vi "ingest.video-with_manifest_timestamp.vi"(6 "Properties and Labels":T1, 7 "Timestamp S3 Path":string, 8 "error in":errorcluster, 9 "Title and Description":cluster{"Title":string, "Description":string}, 10 "S3 Path":string, 11 "Nominal Client in":refnum<class "Nominal Client.lvclass">) -> (0 "error out":errorcluster, 1 "Response":T2, 2 "Video RID":string, 3 "Nominal Client out":refnum<class "Nominal Client.lvclass">, 4 "Response":string)   [LabVIEW 2020, in "Nominal Client.lvclass"]
doc: "Ingests video data from a S3 Nominal upload bucket."
uses:
  Nominal Client.lvclass
  4b965f09-dc68-4d5e-a5c1-32d476accfd4.vi
  1697451f-e5b3-4789-844d-430f2d519a58.vi
  bab285cf-d058-4520-b957-25c58aac0c58.vi
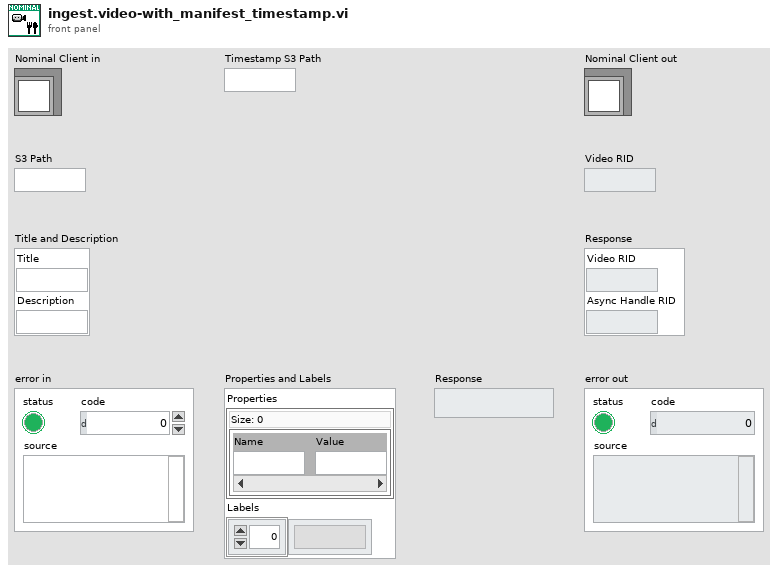
[diagram p1: front panel]
types:
  T1 = cluster{"Properties":map{string, string}, "Labels":string[]}
  T2 = cluster{"Video RID":string, "Async Handle RID":string}
  T3 = cluster{"type":string, "s3":cluster{"path":string}}[]
  T4 = cluster{"type":string, "s3":cluster{"path":string}}
  T5 = cluster{"type":string, "timestampManifests":cluster{"sources":cluster{"type":string, "s3":cluster{"path":string}}[]}}
  T6 = cluster{"videoRid":string, "asyncHandle":cluster{"rid":string}}
  T7 = cluster{"sources":cluster{"type":string, "s3":cluster{"path":string}}[], "properties":string, "labels":string[], "timestamps":cluster{"type":string, "timestampManifests":cluster{"sources":cluster{"type":string, "s3":cluster{"path":string}}[]}}, "title":string, "description":string}
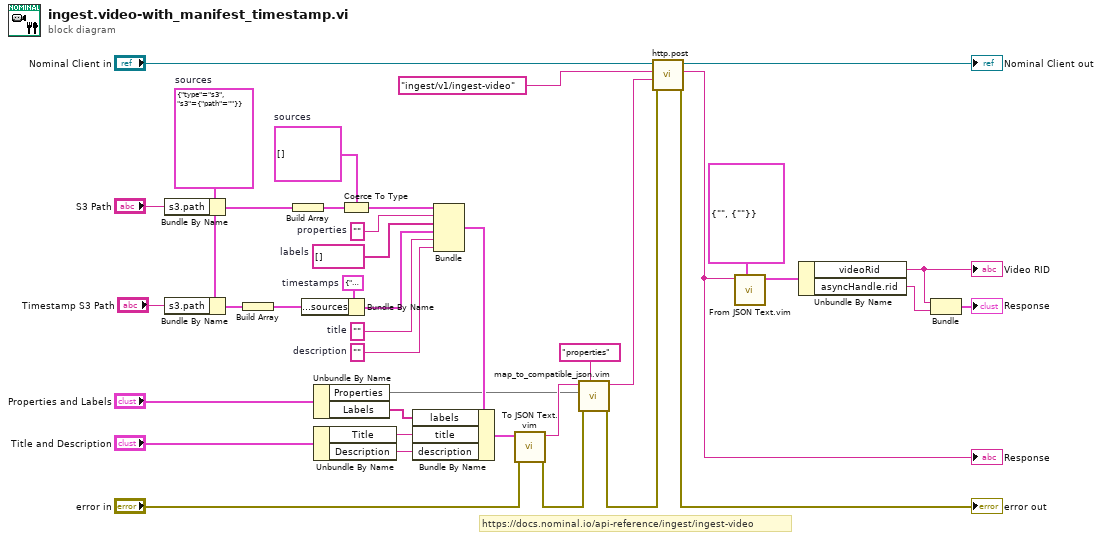
[diagram p0: block diagram]
diagram:
  w9 = T3 []  # sources
  w5 = T4 {"type"="s3", "s3"={"path"=""}}  # sources
  w25 = ""  # description
  w26 = ""  # title
  w3 = T5 {"type"="timestampManifests", "timestampManifests"={"sources"=[]}}  # timestamps
  w27 = string[] []  # labels
  w28 = ""  # properties
  # "https://docs.nominal.io/api-reference/ingest/ingest-video"
  n1 = Bundle By Name(cluster=w5, "s3.path"="S3 Path") -> (w11:T4)
  n2 = Bundle By Name(cluster=w5, "s3.path"="Timestamp S3 Path") -> (w4:T4)
  n3 = Build Array(w4) -> (w2:T3)
  n4 = Build Array(w11) -> (w10:T3)
  n5 = Bundle By Name(cluster=w3, "timestampManifests.sources"=w2) -> (w1:T5)
  n6 = Unbundle By Name("Properties and Labels") -> ("Properties"=w15:map{string, string}, "Labels"=w23:string[])
  n7 = Unbundle By Name("Title and Description") -> ("Title"=w21:string, "Description"=w20:string)
  n8 = Coerce To Type(0:w10, 1:w9) -> (2:w7:T3)
  n9 = Bundle("sources"=w7, "properties"=w28, "labels"=w27, "timestamps"=w1, "title"=w26, "description"=w25) -> (w24:T7)  [unwired: 1 in]
  n10 = Bundle By Name(cluster=w24, "labels"=w23, "title"=w21, "description"=w20) -> (w19:T7)
  n11 = call "To JSON Text.vim"("error in (no error)"="error in", "Anything"=w19) -> ("error out"=w13:errorcluster, "<JSON>"=w16:string)  [unwired: 8 in]
  n12 = call "map_to_compatible_json.vim"("JSON Path"="properties" ("Data Name"), "error in"=w13, "Map"=w15, "JSON in"=w16) -> ("error out"=w12:errorcluster, "JSON out"=w14:string)  [unwired: 6 in]
  n13 = call "http.post.vi"("error in"=w12, "Request body"=w14, "Path"="ingest/v1/ingest-video", "Nominal Client in"="Nominal Client in") -> ("error out"=→"error out":errorcluster, "Response"=w33:string, "Nominal Client out"=→"Nominal Client out":refnum<class "Nominal Client.lvclass">)  [unwired: 4 in, 1 out]
  "Response" <- w33
  n14 = call "From JSON Text.vim"("Data Type and Default Value"=T6 {"videoRid"="", "asyncHandle"={"rid"=""}} ("Information"), "JSON"=w33) -> ("Data out"=w32:T6)  [unwired: 8 in, 1 out]
  n15 = Unbundle By Name(w32) -> ("videoRid"=w31:string, "asyncHandle.rid"=w30:string)
  "Video RID" <- w31
  n16 = Bundle("videoRid"=w31, "rid"=w30) -> (→"Response":cluster{"videoRid":string, "rid":string})  [unwired: 1 in]
